vi "SMTP Email Transliterate Settings.vi"(4 "transliteration":string caption="translittération", 5 "character set":string caption="jeu de caractères") -> (0 "map":u8[](array[numeric]) caption="mappage", 1 "charset out":string caption="jeu de caractères en sortie")   [LabVIEW 2022 SP3, in "Copie de NI_SMTPEmail.lvlib"]
doc: "Ne modifie pas les paramètres par défaut pour les VIs SMTP. Quand fonction est \"utilisation\", toutes les entrées (l'objet, le serveur, l'adresse de retour ou le jeu de caractères) qui ne sont pas vides ne sont pas modifées. Les autres sont remplacées par les paramètres par défaut.\n\nfonction - spécifie l'action à réaliser (par défaut, utilisation).\n utilisation - remplace les entrées vides par les paramètres par défaut et les renvoie dans les sorties adresse de retour, serveur, objet et jeu de caractère. Renvoie également un mappage à appliquer aux messages texte.\n configuration - définit les valeurs par défaut à adresse de retour, objet, serveur et jeu de caractères. Charge aussi les tables de translittération basées sur la translittération.\n lire ini - définit les paramètres par défaut pour le fichier SMTP.ini\n\nadresse de retour - adresse de retour à utiliser (par défaut, celle qui est dans SMTP.ini)\n\nobjet - objet à utiliser (par défaut, celui contenu dans SMTP.ini)\n\nserveur - serveur SMTP à utiliser (par défaut, celui qui est dans SMTP.ini)\n\njeu de caractères - jeu de caractères à utiliser (par défaut, celui contenu dans SMTP.ini)\n\ntranslittération - (avec configuration) spécifie quelles sont les tables de translittération à charger\n\nmap - (avec utilisation) spécifie comment les caractères doivent être mappés."
uses:
  Copie de NI_SMTPEmail.lvlib
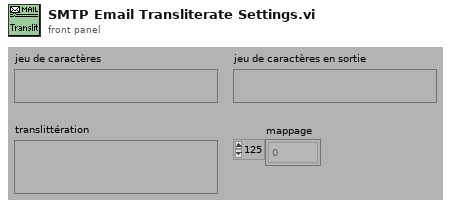
[diagram p1: front panel]
types:
  T1 = typedef "Copie de NI_SMTPEmail.lvlib/SMTP Email Keyed Array.ctl" = cluster{"keys":string[], "values":string[]}
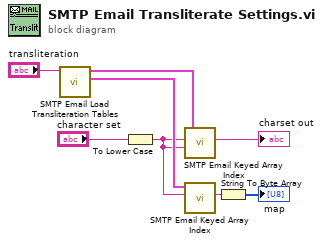
[diagram p0: block diagram]
diagram:
  n1 = call "SMTP Email Load Transliteration Tables.vi"("\"Transliterate\" config"="transliteration") -> ("maps"=w6:T1, "charsets"=w7:T1)  [unwired: 5 in]
  n2 = To Lower Case(string="character set") -> (all lower case string=w2:string)
  n3 = call "SMTP Email Keyed Array Index.vi"("default value"=w2, "key"=w2, "array in"=w7) -> ("value"=→"charset out":string)  [unwired: 2 in, 2 out]
  n4 = call "SMTP Email Keyed Array Index.vi"("key"=w2, "array in"=w6) -> ("value"=w5:string)  [unwired: 3 in, 2 out]
  n5 = String To Byte Array(string=w5) -> (unsigned byte array=→"map":u8[])
